vi "Get Owning Project.vi"(7 "VI":refnum<vi>, 8 "error in":errorcluster) -> (0 "error out":errorcluster, 2 "Owning Project":refnum<vi>)   [LabVIEW 2020]
doc: "Gets a reference to the opened project that owns the VI. The project is then traversed to verify the VI is explicitly part of the project (not in Dependencies or just in memory)."
panel:
  out "Non-qualified Name":string
  out "VI Found":bool
  out "Project Name":string
  out "VI Name":string
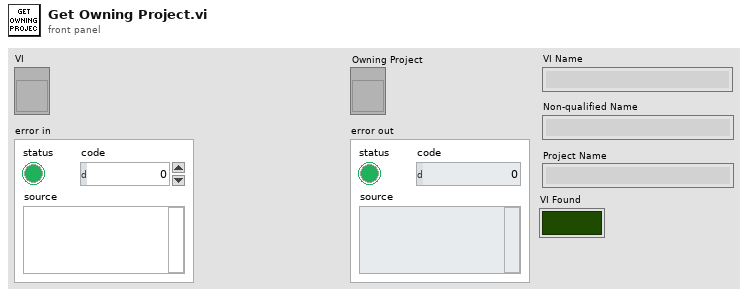
[diagram p1: front panel]
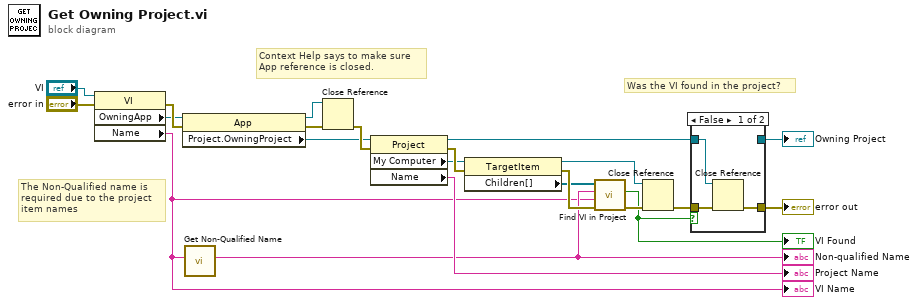
[diagram p0: block diagram]
diagram:
  # "The Non-Qualified name is required due to the project item names"
  # "Was the VI found in the project?"
  # "Context Help says to make sure App reference is closed."
  n1 = property class="VI"(reference="VI", error in="error in") -> (error out=w21:errorcluster, "OwningApp"=w11:refnum<vi>, "Name"=w2:string)  [unwired: 1 out]
  "VI Name" <- w2
  n2 = property class="App"(reference=w11, error in=w21) -> (reference out=w12:refnum<vi>, error out=w22:errorcluster, "Project.OwningProject"=w7:refnum<vi>)
  n3 = call "Get Non-Qualified Name.vi"("VI Name"=w2) -> ("Non-Qualified VI Name"=w3:string)  [unwired: 10 in]
  "Non-qualified Name" <- w3
  n4 = Close Reference(reference=w12, error in (no error)=w22) -> (error out=w17:errorcluster)
  n5 = property class="Project"(reference=w7, error in=w17) -> (reference out=w5:refnum<vi>, error out=w18:errorcluster, "My Computer"=w10:refnum<vi>, "Name"=→"Project Name":string)
  n6 = property class="TargetItem"(reference=w10, error in=w18) -> (reference out=w1:refnum<vi>, error out=w19:errorcluster, "Children[]"=w8:refnum<vi>[])
  n7 = call "Find VI in Project.vi"("error in"=w19, "VI Name"=w2, "Non-Qualified VI Name"=w3, "Project Items"=w8) -> ("error out"=w15:errorcluster, "VI Found"=w6:bool)  [unwired: 6 in]
  "VI Found" <- w6
  n8 = Close Reference(reference=w1, error in (no error)=w15) -> (error out=w14:errorcluster)
  n9 = case shown="False" w6 {
    tunnel: w5 -> [w23 w26]
    tunnel: w14 -> [w25 w27]
    tunnel: [w24 w27] -> w16
    tunnel: [_ w26] -> w4
    frame False {
      n10 = Close Reference(reference=w23, error in (no error)=w25) -> (error out=w24:errorcluster)
    }
    frame True {
    }
  }
  "Owning Project" <- w4
  "error out" <- w16
